vi "CIF Publisher to Refnum.vi"(3 "CIF Publisher U64":u64) -> (5 "CIF Publisher Refnum":T1 {"refnum" format="%.0x"})   [LabVIEW 2021, in "Iceoryx.lvlib"]
uses:
  Iceoryx.lvlib
  Typedef/CIF Publisher Refnum.ctl
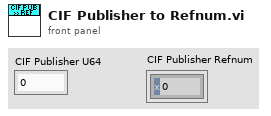
[diagram p1: front panel]
types:
  T1 = typedef "Iceoryx.lvlib/CIF Publisher Refnum.ctl" = cluster{"refnum":u64, "CIF Pub":enum8{"cifpub"}}
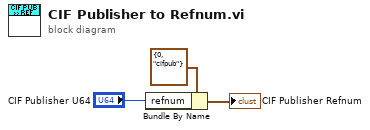
[diagram p0: block diagram]
diagram:
  n1 = Bundle By Name(cluster=T1 {"refnum"=0, "CIF Pub"=enum."cifpub"} ("CIF Publisher Refnum"), "refnum"="CIF Publisher U64") -> (→"CIF Publisher Refnum":T1)
